vi "Write Name.vi"(8 "error in (no error)":errorcluster, 10 "Name":string, 11 "Gauge in":refnum<class "Gauge.lvclass">) -> (0 "error out":errorcluster, 3 "Gauge out":refnum<class "Gauge.lvclass">)   [LabVIEW 2026, in "Gauge.lvclass"]
doc: "Writes one field of this class's private data. Generated by lvai_create_accessors from the class private data control."
uses:
  Gauge.lvclass
  Gauge.lvclass/Gauge.ctl
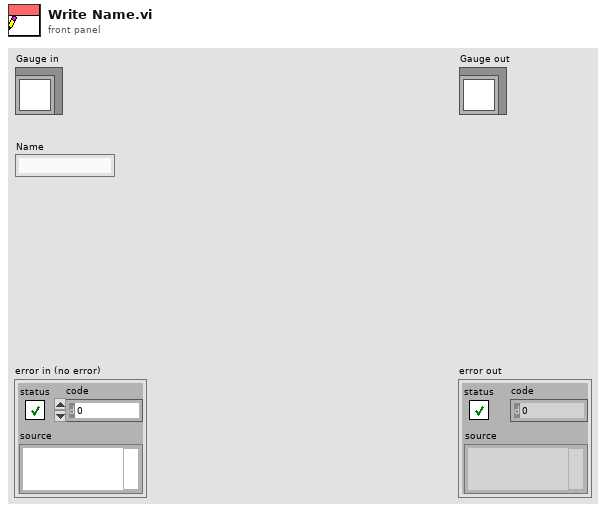
[diagram p1: front panel]
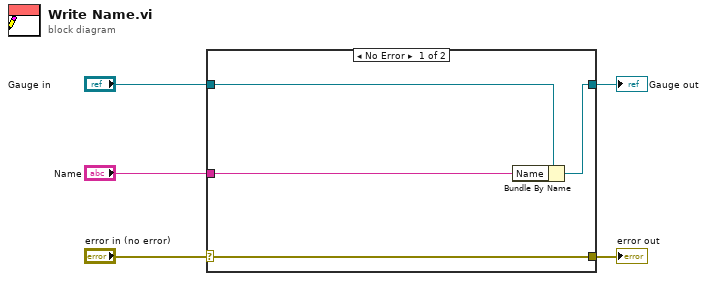
[diagram p0: block diagram]
diagram:
  n1 = case shown="No Error" "error in (no error)" {
    selector: "error in (no error)" -> [w9 w10]
    tunnel: [w9 w10] -> w4
    tunnel: [w7 w11] -> w2
    tunnel: "Gauge in" -> [w8 w11]
    tunnel: "Name" -> [w6 _]
    frame No Error {
      n2 = Bundle By Name(cluster=w8, "Name"=w6) -> (w7:refnum<class "Gauge.lvclass">)
    }
    frame Error {
    }
  }
  "error out" <- w4
  "Gauge out" <- w2
